vi "VM Spy - create context.vi"() -> (0 "OK out":bool, 3 "VC Handle out":T1=-1)   [LabVIEW 2021]
doc: "::: CalcExpress Toolkit :::\nCopyright (c) 2000-2026 Konstantin Shifershteyn. All rights reserved."
uses:
  vi.lib/addons/CalcExpress/cetypes.llb/VarMan Variable Context Handle.ctl
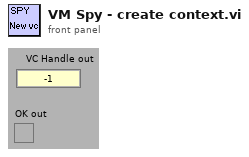
[diagram p1: front panel]
types:
  T1 = typedef "VarMan Variable Context Handle.ctl" = i32
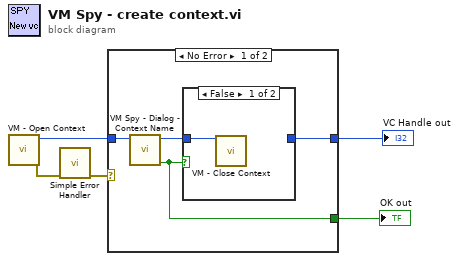
[diagram p0: block diagram]
diagram:
  n1 = call "VM - Open Context.vi"() -> ("error out"=w4:errorcluster, "VC Handle out"=w5:T1)  [unwired: 9 in, 1 out]
  n2 = call <vilib>:"Simple Error Handler.vi"("error in (no error)"=w4) -> ("error out"=w3:errorcluster)  [unwired: 4 in, 4 out]
  n3 = case shown="No Error" w3 {
    tunnel: w5 -> [w9 _]
    tunnel: [w7 _] -> w2
    tunnel: [w6 _] -> w1
    frame No Error {
      n4 = call "VM Spy - Dialog - Context Name.vi"("VC Handle"=w9) -> ("OK out"=w6:bool, "dup VC Handle"=w8:T1)  [unwired: 9 in]
      n5 = case shown="False" w6 {
        tunnel: w8 -> [w10 w11]
        tunnel: [_ w11] -> w7
        frame False {
          n6 = call "VM - Close Context.vi"("VC Handle"=w10) -> ()  [unwired: 9 in, 2 out]
        }
        frame True {
        }
      }
    }
    frame Error {
    }
  }
  "OK out" <- w1
  "VC Handle out" <- w2
